vi "pull data from point buffer.vi"(11 "point buffer":refnum<data-value>) -> (0 "error out":errorcluster, 3 "data value":T1)   [LabVIEW 2020, in "nominal core steps.lvlib"]
doc: "Reads the entire set of samples from a buffer."
uses:
  nominal core steps.lvlib
  points buffer.ctl
  single point.ctl
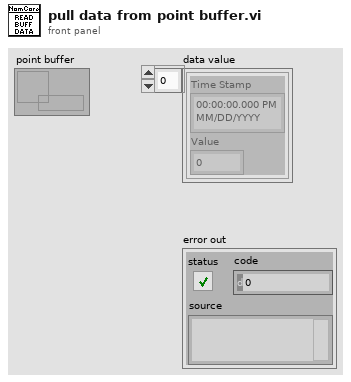
[diagram p1: front panel]
types:
  T1 = typedef "nominal core steps.lvlib/points buffer.ctl" = T2[]
  T2 = typedef "nominal core steps.lvlib/single point.ctl" = cluster{"Time Stamp":timestamp, "Value":dbl}
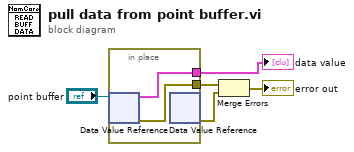
[diagram p0: block diagram]
diagram:
  n1 = in-place {
    in-place-border: [w7] -> w3
    in-place-border: [w6] -> w1
    n2 = in-place-dvr #1("point buffer") -> (w6:T1, w7:errorcluster)
    n3 = in-place-dvr #1() -> (w4:errorcluster)  [unwired: 1 in, 1 out]
  }
  "data value" <- w1
  n4 = Merge Errors(w3, w4) -> (→"error out":errorcluster)
